vi "SUP_Camera_Transport.vi"() -> ()   [LabVIEW 2012]
panel:
  out "Queue cleanup error 2":errorcluster caption="sortie d'erreur"
  out "Queue cleanup error":errorcluster caption="sortie d'erreur"
  in  "packet":variant
  in  "Stop telemetry transport":bool
  out "Ack length in range (required)":bool
  out "Telemetry transport error only":errorcluster caption="sortie d'erreur"
  out "Ack JSON (raw; not validated)":string
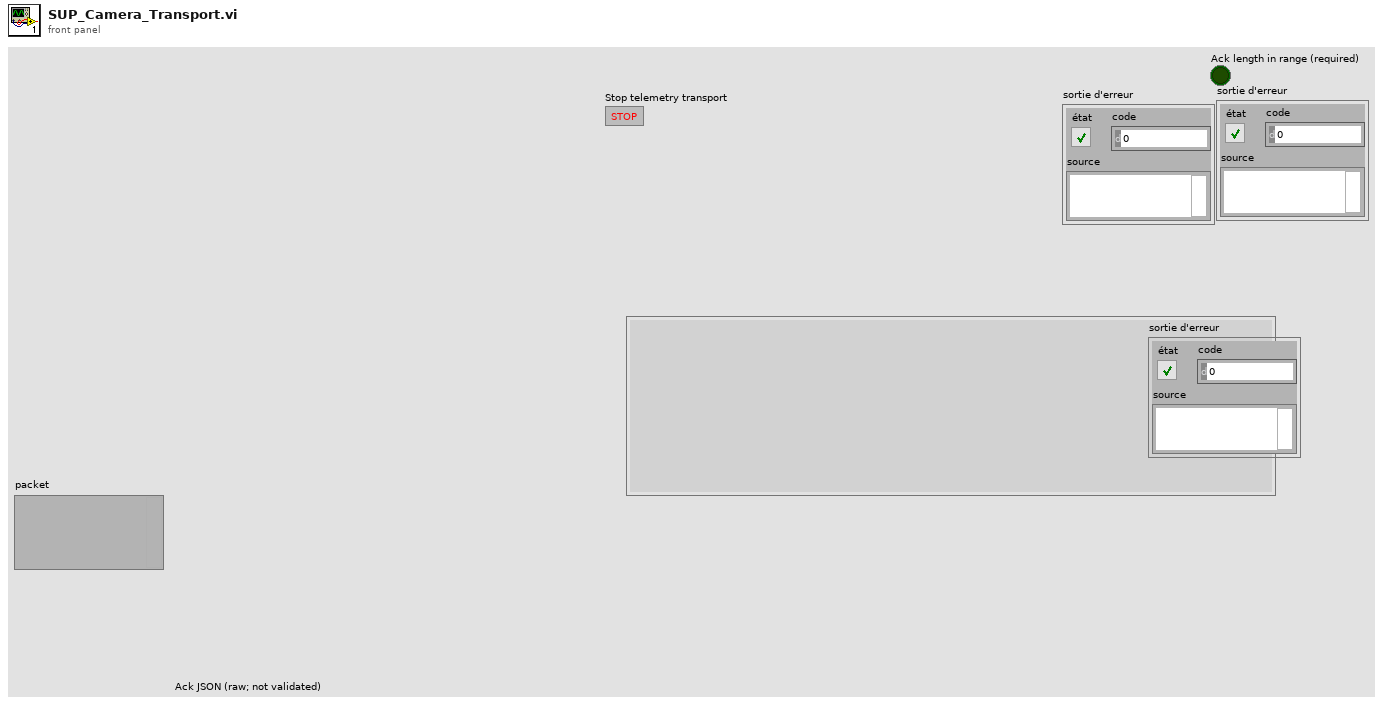
[diagram p1: front panel]
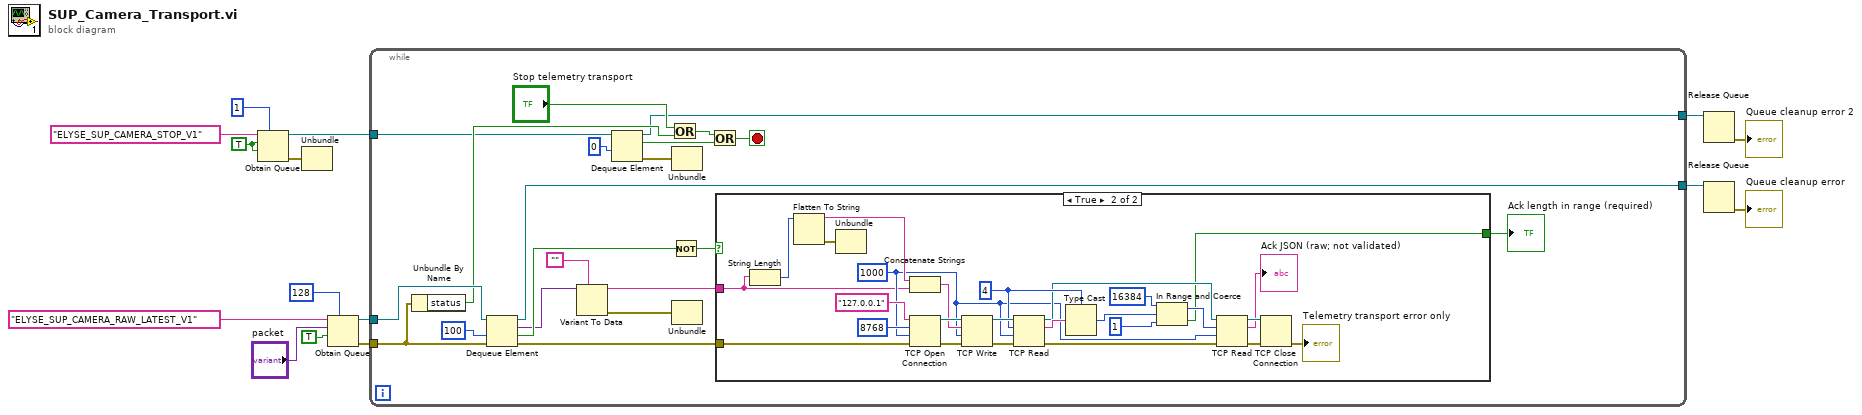
[diagram p0: block diagram]
diagram:
  w6 = TRUE ("créer si introuvable ? (V)")
  n1 = Obtain Queue(max queue size (-1, unlimited)=1 ("taille max de la file d'attente (-1, non limitée)"), name (unnamed)="ELYSE_SUP_CAMERA_STOP_V1" ("nom (aucun)"), element data type=w6, create if not found? (T)=w6) -> (queue out=w5:refnum<queue>, error out=w1:errorcluster)  [unwired: 1 in, 1 out]
  n2 = Unbundle(w1) -> ()  [unwired: 3 out]
  n3 = Obtain Queue(max queue size (-1, unlimited)=128 ("taille max de la file d'attente (-1, non limitée)"), name (unnamed)="ELYSE_SUP_CAMERA_RAW_LATEST_V1" ("nom (aucun)"), element data type="packet", create if not found? (T)=TRUE ("créer si introuvable ? (V)")) -> (queue out=w12:refnum<queue>, error out=w11:errorcluster)  [unwired: 1 in, 1 out]
  n4 = while {
    tunnel: w12 -> [w35]
    tunnel: w11 -> [w31]
    tunnel: [w32] -> w10
    tunnel: w5 -> [w25]
    tunnel: [w21] -> w3
    stop <- w22 stop-if-true
    n5 = Unbundle By Name(w31) -> ("status"=w29:bool)
    n6 = Dequeue Element(queue=w35, timeout in ms (-1)=100 ("timeout en ms (-1)"), error in (no error)=w31) -> (queue out=w32:refnum<queue>, element=w19:variant, timed out?=w28:bool, error out=w33:errorcluster)
    n7 = Variant To Data(type="", Variant=w19) -> (data=w18:string, error out=w17:errorcluster)  [unwired: 1 in]
    n8 = Dequeue Element(queue=w25, timeout in ms (-1)=0 ("timeout en ms (-1)")) -> (queue out=w21:refnum<queue>, element=w23:bool, error out=w16:errorcluster)  [unwired: 1 in, 1 out]
    n9 = Or(x="Stop telemetry transport", y=w29) -> (x .or. y?=w24:bool)
    n10 = Not(x=w28) -> (.not. x?=w27:bool)
    n11 = Unbundle(w16) -> ()  [unwired: 3 out]
    n12 = Unbundle(w17) -> ()  [unwired: 3 out]
    n13 = Or(x=w24, y=w23) -> (x .or. y?=w22:bool)
    n14 = case shown="True" w27 {
      tunnel: [_ w40] -> w36
      tunnel: w33 -> [_ w39]
      tunnel: w18 -> [_ w38]
      frame False {
      }
      frame True {
        w43 = 1000 ("timeout en ms (60000)")
        w53 = 4 ("octets à lire")
        n15 = String Length(string=w38) -> (length=w58:i32)
        n16 = Flatten To String(anything=w58) -> (data string=w57:string, error out=w37:errorcluster)  [unwired: 3 in, 1 out]
        n17 = Unbundle(w37) -> ()  [unwired: 3 out]
        n18 = Concatenate Strings(w57, w38) -> (w56:string)
        n19 = TCP Open Connection(address="127.0.0.1" ("adresse"), remote port or service name=u16 8768 ("port distant ou nom du service"), timeout ms (60000)=w43, error in (no error)=w39) -> (connection ID=w60:refnum<k5>, error out=w59:errorcluster)  [unwired: 1 in]
        n20 = TCP Write(connection ID=w60, data in=w56, error in (no error)=w59, 9:w43) -> (connection ID out=w55:refnum<k5>, error out=w54:errorcluster)  [unwired: 1 out]
        n21 = TCP Read(connection ID=w55, bytes to read=w53, error in (no error)=w54, 9:w43) -> (connection ID out=w51:refnum<k5>, data out=w52:string, error out=w50:errorcluster)  [unwired: 1 in]
        n22 = Type Cast(type=w53, x=w52) -> (*(type *) &x=w49:i32)
        n23 = In Range and Coerce(upper limit=16384 ("limite supérieure"), x=w49, lower limit=1 ("limite inférieure")) -> (coerced(x)=w46:i32, In Range?=w40:bool)
        n24 = TCP Read(connection ID=w51, bytes to read=w46, error in (no error)=w50, 9:w43) -> (connection ID out=w45:refnum<k5>, data out=→"Ack JSON (raw; not validated)":string, error out=w44:errorcluster)  [unwired: 1 in]
        n25 = TCP Close Connection(connection ID=w45, error in (no error)=w44) -> (error out=→"Telemetry transport error only":errorcluster)  [unwired: 1 in, 1 out]
      }
    }
    "Ack length in range (required)" <- w36
  }
  n26 = Release Queue(queue=w3) -> (error out=→"Queue cleanup error 2":errorcluster)  [unwired: 2 in, 2 out]
  n27 = Release Queue(queue=w10) -> (error out=→"Queue cleanup error":errorcluster)  [unwired: 2 in, 2 out]
